vi "Set ConfigFile.vi"(8 "error in (no error)":errorcluster, 11 "Plugins Folder":path) -> (0 "error out":errorcluster)   [LabVIEW 2021, in "Channel.lvlib"]
uses:
  Channel.lvlib
  Private/G_Paths.vi
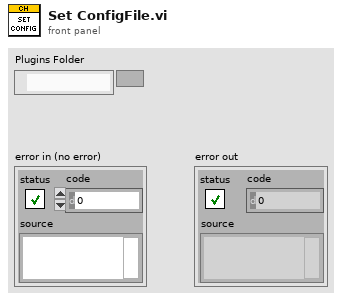
[diagram p1: front panel]
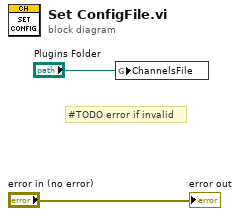
[diagram p0: block diagram]
diagram:
  # "#TODO error if invalid"
  n1 = global write "G_Paths.vi" "ChannelsFile"("Plugins Folder") -> ()
  "error out" <- "error in (no error)"
